vi "Compare results.vi"(0 "string":string, 5 "Boolean":bool, 11 "?":errorcluster) -> (3 "Result":bool, 4 "Current":string, 6 "Measured Voltage":string, 8 "Result":string, 15 "?":errorcluster)   [LabVIEW 2021]
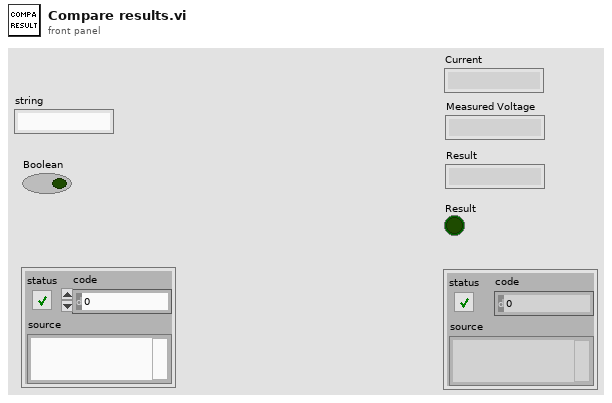
[diagram p1: front panel]
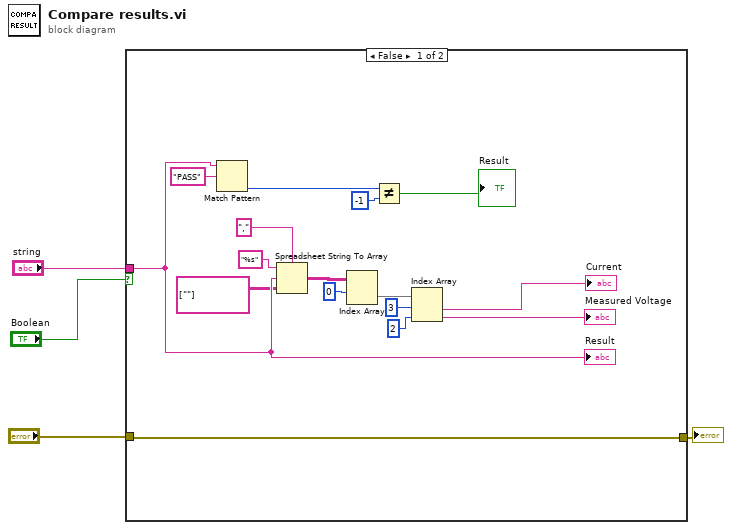
[diagram p0: block diagram]
diagram:
  n1 = case shown="False" "Boolean" {
    tunnel: "string" -> [w20 _]
    tunnel: "?" -> [w5 w21]
    tunnel: [w5 w21] -> w2
    frame False {
      n2 = Match Pattern(string=w20, regular expression="PASS") -> (offset past match=w17:i32)  [unwired: 1 in, 3 out]
      n3 = Spreadsheet String To Array(delimiter (Tab)=",", format string="%s", spreadsheet string=w20, array type (2D Dbl)=string[][] [[""]]) -> (array=w12:string[][])
      n4 = Index Array(array=w12, index (row)=0) -> (element=w10:string[])  [unwired: 1 in]
      n5 = Not Equal?(x=w17, y=-1) -> (x != y?=→"Result":bool)
      n6 = Index Array(array=w10, index #1=3 ("index"), index #2=2 ("index")) -> (element #1=→"Current":string, element #2=→"Measured Voltage":string)
      "Result" <- w20
    }
    frame True {
    }
  }
  "?" <- w2
